vi "lvmcp_uids.vi"() -> ()   [LabVIEW 2026]
uses:
  <vilib>/Utility/traverseref.llb/TRef TravTarget.ctl
panel:
  out "Values":variant[](array[variant])
  out "Names":string[](array[string])
  out "Wire UIDs":i32[](array[numeric])
  out "Is Source":bool[](array[boolean])
  out "Owner UIDs":i32[](array[numeric])
  in  "Traverse Target":T1
  out "References":refnum<vi>[](array[refnum])
  out "Classes":string[](array[string])
  out "UIDs":i32[](array[numeric])
  in  "error in (no error)":errorcluster
  in  "Class Name":string
  in  "VI Refnum":refnum<vi>
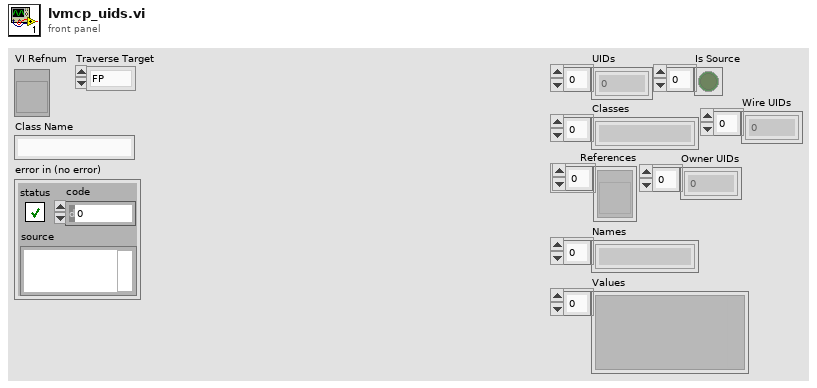
[diagram p1: front panel]
types:
  T1 = typedef "TRef TravTarget.ctl" = enum16{"FP", "BD", "Other"}
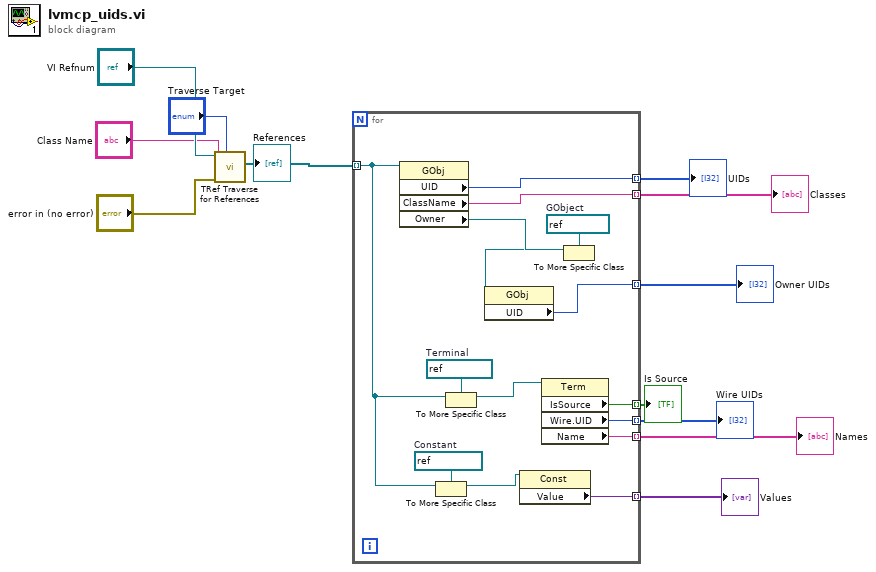
[diagram p0: block diagram]
diagram:
  n1 = call <vilib>:"TRef Traverse for References.vi"("Traverse Target"="Traverse Target", "error in (no error)"="error in (no error)", "Class Name"="Class Name", "VI Refnum"="VI Refnum") -> ("References"=w7:refnum<vi>[])  [unwired: 4 in, 3 out]
  "References" <- w7
  n2 = for {
    tunnel: [w27] -> w9 mode=indexing
    tunnel: [w26] -> w8 mode=indexing
    tunnel: w7 -> [w16] mode=indexing
    tunnel: [w22] -> w5 mode=indexing
    tunnel: [w19] -> w4 mode=indexing
    tunnel: [w18] -> w3 mode=indexing
    tunnel: [w17] -> w2 mode=indexing
    tunnel: [w13] -> w1 mode=indexing
    w15 = refnum<vi> refnum  # Constant
    w21 = refnum<vi> refnum  # Terminal
    w24 = refnum<vi> refnum  # GObject
    n3 = property class="GObj"(reference=w16) -> ("UID"=w26:i32, "ClassName"=w27:string, "Owner"=w25:refnum<vi>)  [unwired: 1 in, 2 out]
    n4 = To More Specific Class(target class=w15, reference=w16) -> (specific class reference=w14:refnum<vi>)  [unwired: 1 in, 1 out]
    n5 = To More Specific Class(target class=w21, reference=w16) -> (specific class reference=w20:refnum<vi>)  [unwired: 1 in, 1 out]
    n6 = property class="Const"(reference=w14) -> ("Value"=w13:variant)  [unwired: 1 in, 2 out]
    n7 = property class="Term"(reference=w20) -> ("IsSource"=w19:bool, "Wire.UID"=w18:i32, "Name"=w17:string)  [unwired: 1 in, 2 out]
    n8 = To More Specific Class(target class=w24, reference=w25) -> (specific class reference=w23:refnum<vi>)  [unwired: 1 in, 1 out]
    n9 = property class="GObj"(reference=w23) -> ("UID"=w22:i32)  [unwired: 1 in, 2 out]
  }
  "UIDs" <- w8
  "Classes" <- w9
  "Owner UIDs" <- w5
  "Is Source" <- w4
  "Wire UIDs" <- w3
  "Names" <- w2
  "Values" <- w1
